vi "RDB Init New Message.vi"(7 "RDB Receive Reference.RDB Signals":dbl[](array[numeric]), 8 "error in (no error)":errorcluster, 9 "Status_Cluster":T1={"simTime"=0.0, "simFrame"=0.0, "Connection Status"=enum."Disconnected", "Connection Command"=enum."Disconnect", "Last Error"=0, "Case selection"=enum."Connecting"}, 10 "RDB Reference in":T7, 11 "Settings in":T4={"UDP Receiver"=refnum, "UDP Sender"=refnum, "Valid Packet"=FALSE, "TCP"=refnum, "Network Settings"={"IP adress"="127.0.0.1", "RDB"={"Protocol"=enum."UDP", "Tx Port"=48270, "Rx Port"=10, "Buffer Size"=204800, "Timeout"=10}, "SCP"={"Protocol"=enum."TCP", "Tx Port"=48191, "Rx Port"=48191, "Buffer Size"=204800, "Timeout"=10}}, "vclient"=path "", "paeseHandle"=0, "builderHandle"=0}) -> (0 "error out":errorcluster, 2 "RDB Reference out":T7, 3 "Settings out":T4={"UDP Receiver"=refnum, "UDP Sender"=refnum, "Valid Packet"=FALSE, "TCP"=refnum, "Network Settings"={"IP adress"="127.0.0.1", "RDB"={"Protocol"=enum."UDP", "Tx Port"=48270, "Rx Port"=10, "Buffer Size"=204800, "Timeout"=10}, "SCP"={"Protocol"=enum."TCP", "Tx Port"=48191, "Rx Port"=48191, "Buffer Size"=204800, "Timeout"=10}}, "vclient"=path "", "paeseHandle"=0, "builderHandle"=0})   [LabVIEW 2023, in "RDB.lvlib"]
uses:
  RDB.lvlib
  RDB References.ctl
  DataContainer/DataContainer.lvclass
  Engine/Type/Settings.ctl
  Shared/Network Settings.ctl
  Shared/Protocol.ctl
  Engine/Type/Status_Cluster.ctl
  Engine/Type/ConnectionStatus.ctl
  Engine/Type/CaseSelection.ctl
  <vilib>/xnet/xnet.llb/XNET Convert (Signal to Frame FlexRay).vi
  Shared/Vires VTD Shared.lvlib
  Engine/Vires VTD Engine.lvlib
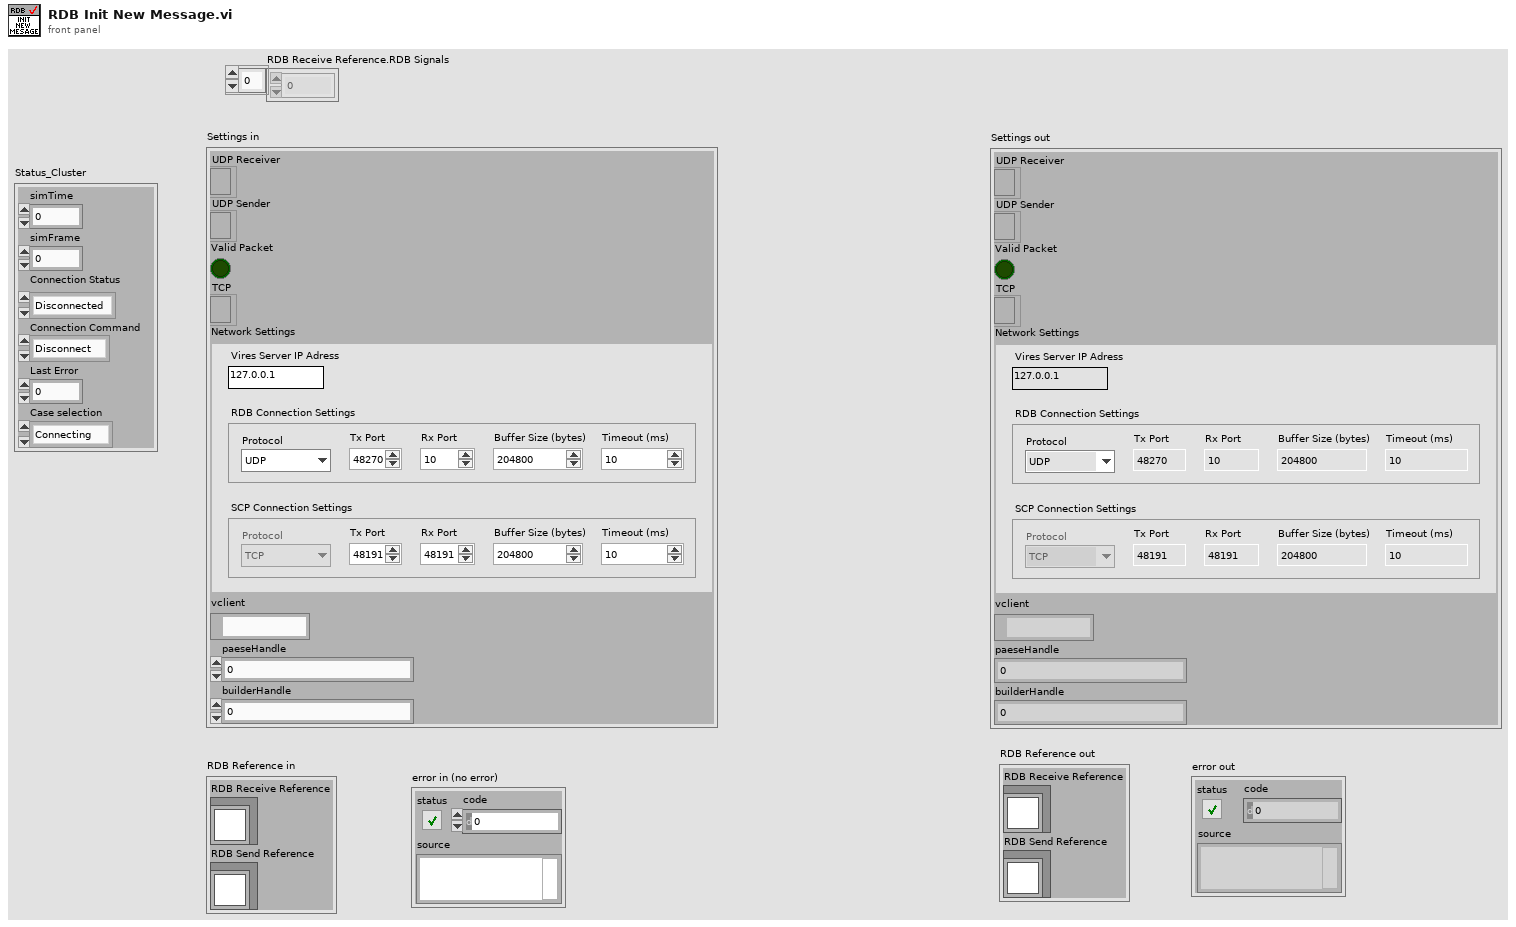
[diagram p1: front panel]
types:
  T1 = typedef "Vires VTD Engine.lvlib/Status_Cluster.ctl" = cluster{"simTime":dbl, "simFrame":dbl, "Connection Status":T2, "Connection Command":enum16{"Disconnect", "Connect"}, "Last Error":i32, "Case selection":T3}
  T2 = typedef "Vires VTD Engine.lvlib/ConnectionStatus.ctl" = enum16{"Disconnected", "Connected"}
  T3 = typedef "Vires VTD Engine.lvlib/CaseSelection.ctl" = enum32{"Idle", "Connecting", "Disconnecting", "Read/Write"}
  T4 = typedef "Vires VTD Engine.lvlib/Settings.ctl" = cluster{"UDP Receiver":refnum<k16>, "UDP Sender":refnum<k16>, "Valid Packet":bool, "TCP":refnum<k5>, "Network Settings":T5, "vclient":path, "paeseHandle":u64, "builderHandle":u64}
  T5 = typedef "Vires VTD Shared.lvlib/Network Settings.ctl" = cluster{"IP adress":string, "RDB":cluster{"Protocol":T6, "Tx Port":u16, "Rx Port":u16, "Buffer Size":i32, "Timeout":u16}, "SCP":cluster{"Protocol":T6, "Tx Port":u16, "Rx Port":u16, "Buffer Size":i32, "Timeout":u16}}
  T6 = typedef "Vires VTD Shared.lvlib/Protocol.ctl" = enum16{"UDP", "TCP"}
  T7 = typedef "RDB.lvlib/RDB References.ctl" = cluster{"RDB Receive Reference":refnum<class "DataContainer.lvclass">, "RDB Send Reference":refnum<class "DataContainer.lvclass">}
  T8 = typedef "XNET Frame FlexRay.ctl" = cluster{"timestamp":timestamp, "payload":u8[], "slot":u16, "type":T9, "cycle count":u8, "startup?":bool, "sync?":bool, "preamble?":bool, "ch A":bool, "ch B":bool, "echo?":bool}
  T9 = typedef "XNET Frame Type FlexRay.ctl" = u8
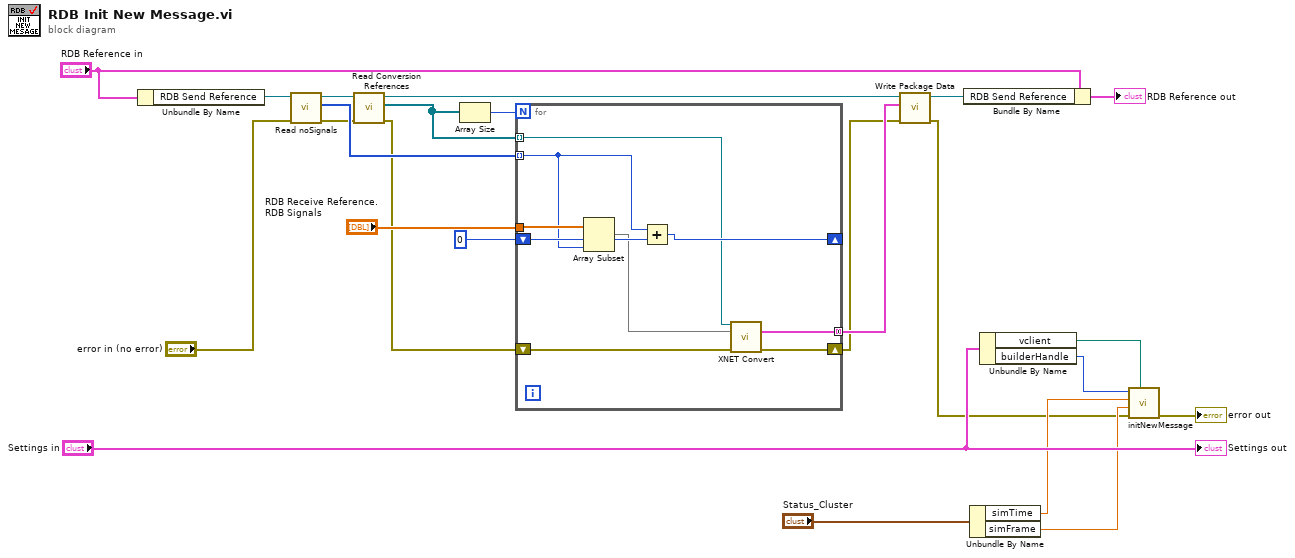
[diagram p0: block diagram]
diagram:
  n1 = Unbundle By Name("RDB Reference in") -> ("RDB Send Reference"=w12:refnum<class "DataContainer.lvclass">)
  n2 = call-dynamic "Read noSignals.vi"("error in (no error)"="error in (no error)", "DataContainer in"=w12) -> ("error out"=w7:errorcluster, "noSignals"=w9:i32[], "DataContainer out"=w11:refnum<class "DataContainer.lvclass">)  [unwired: 7 in]
  n3 = call-dynamic "Read Conversion References.vi"("error in (no error)"=w7, "DataContainer in"=w11) -> ("error out"=w6:errorcluster, "Conversion References"=w10:refnum<k21>[], "DataContainer out"=w4:refnum<class "DataContainer.lvclass">)  [unwired: 7 in]
  n4 = Array Size(array=w10) -> (size(s)=w23:i32)
  n5 = for {
    N: w23 -> [_]
    shift-right: [w29] -> w3
    shift-left: w6 -> [w26]
    tunnel: w10 -> [w27] mode=indexing
    tunnel: "RDB Receive Reference.RDB Signals" -> [w33]
    shift-right: [w31] -> _
    shift-left: 0 -> [w32]
    tunnel: [w28] -> w5 mode=concatenating
    tunnel: w9 -> [w25] mode=indexing
    n6 = Array Subset(array=w33, index=w32, length=w25) -> (w30:dbl[])
    n7 = Add(x=w25, y=w32) -> (x+y=w31:i32)
    n8 = call-poly <vilib>:"XNET Convert.vi"("session in"=w27, "signal data"=w30, "error in (no error)"=w26) -> ("frame data"=w28:T8[], "error out"=w29:errorcluster)  [unwired: 9 in, 2 out]
  }
  n9 = call-dynamic "Write Package Data.vi"("error in (no error)"=w3, "Package Data"=w5, "DataContainer in"=w4) -> ("error out"=w1:errorcluster, "DataContainer out"=w2:refnum<class "DataContainer.lvclass">)  [unwired: 7 in]
  n10 = Bundle By Name(cluster="RDB Reference in", "RDB Send Reference"=w2) -> (→"RDB Reference out":T7)
  n11 = Unbundle By Name("Status_Cluster") -> ("simTime"=w15:dbl, "simFrame"=w14:dbl)
  n12 = Unbundle By Name("Settings in") -> ("vclient"=w19:path, "builderHandle"=w17:u64)
  n13 = call "initNewMessage.vi"("path in"=w19, "error in (no error)"=w1, "simFrame"=w14, "simTime"=w15, "builderHandle in"=w17) -> ("error out"=→"error out":errorcluster)  [unwired: 5 in, 1 out]
  "Settings out" <- "Settings in"
